vi "Handmatige besturing met druksensoruitlezing Herschreven.vi"() -> ()   [LabVIEW 2024]
uses:
  <vilib>/DAQmx/write.llb/DAQmx Write (Digital 1D Bool NChan 1Samp 1Line).vi
  <vilib>/DAQmx/read.llb/DAQmx Read (Analog 1D DBL NChan 1Samp).vi
  <vilib>/DAQmx/write.llb/DAQmx Write (Analog DBL 1Chan 1Samp).vi
  <vilib>/DAQmx/create/channels.llb/DAQmx Create Channel (AO-Voltage-Basic).vi
  <vilib>/DAQmx/miscellaneous.llb/DAQmx Fill In Error Info.vi
panel:
  out "Waveform Chart":T1(graph)
  out "data":dbl[](array[numeric]) format="%#_6p"
  out "x-y":dbl
  out "Waveform Chart 2":waveform(dbl)[](graph)
  in  "stop":bool
  in  "file path":path
  in  "Analog output pressure regulator":tag="Dev1/ao0"
  in  "Set pressure Hybrid Heart (Bar)":dbl min=0.0 max=1.0 step=0.1
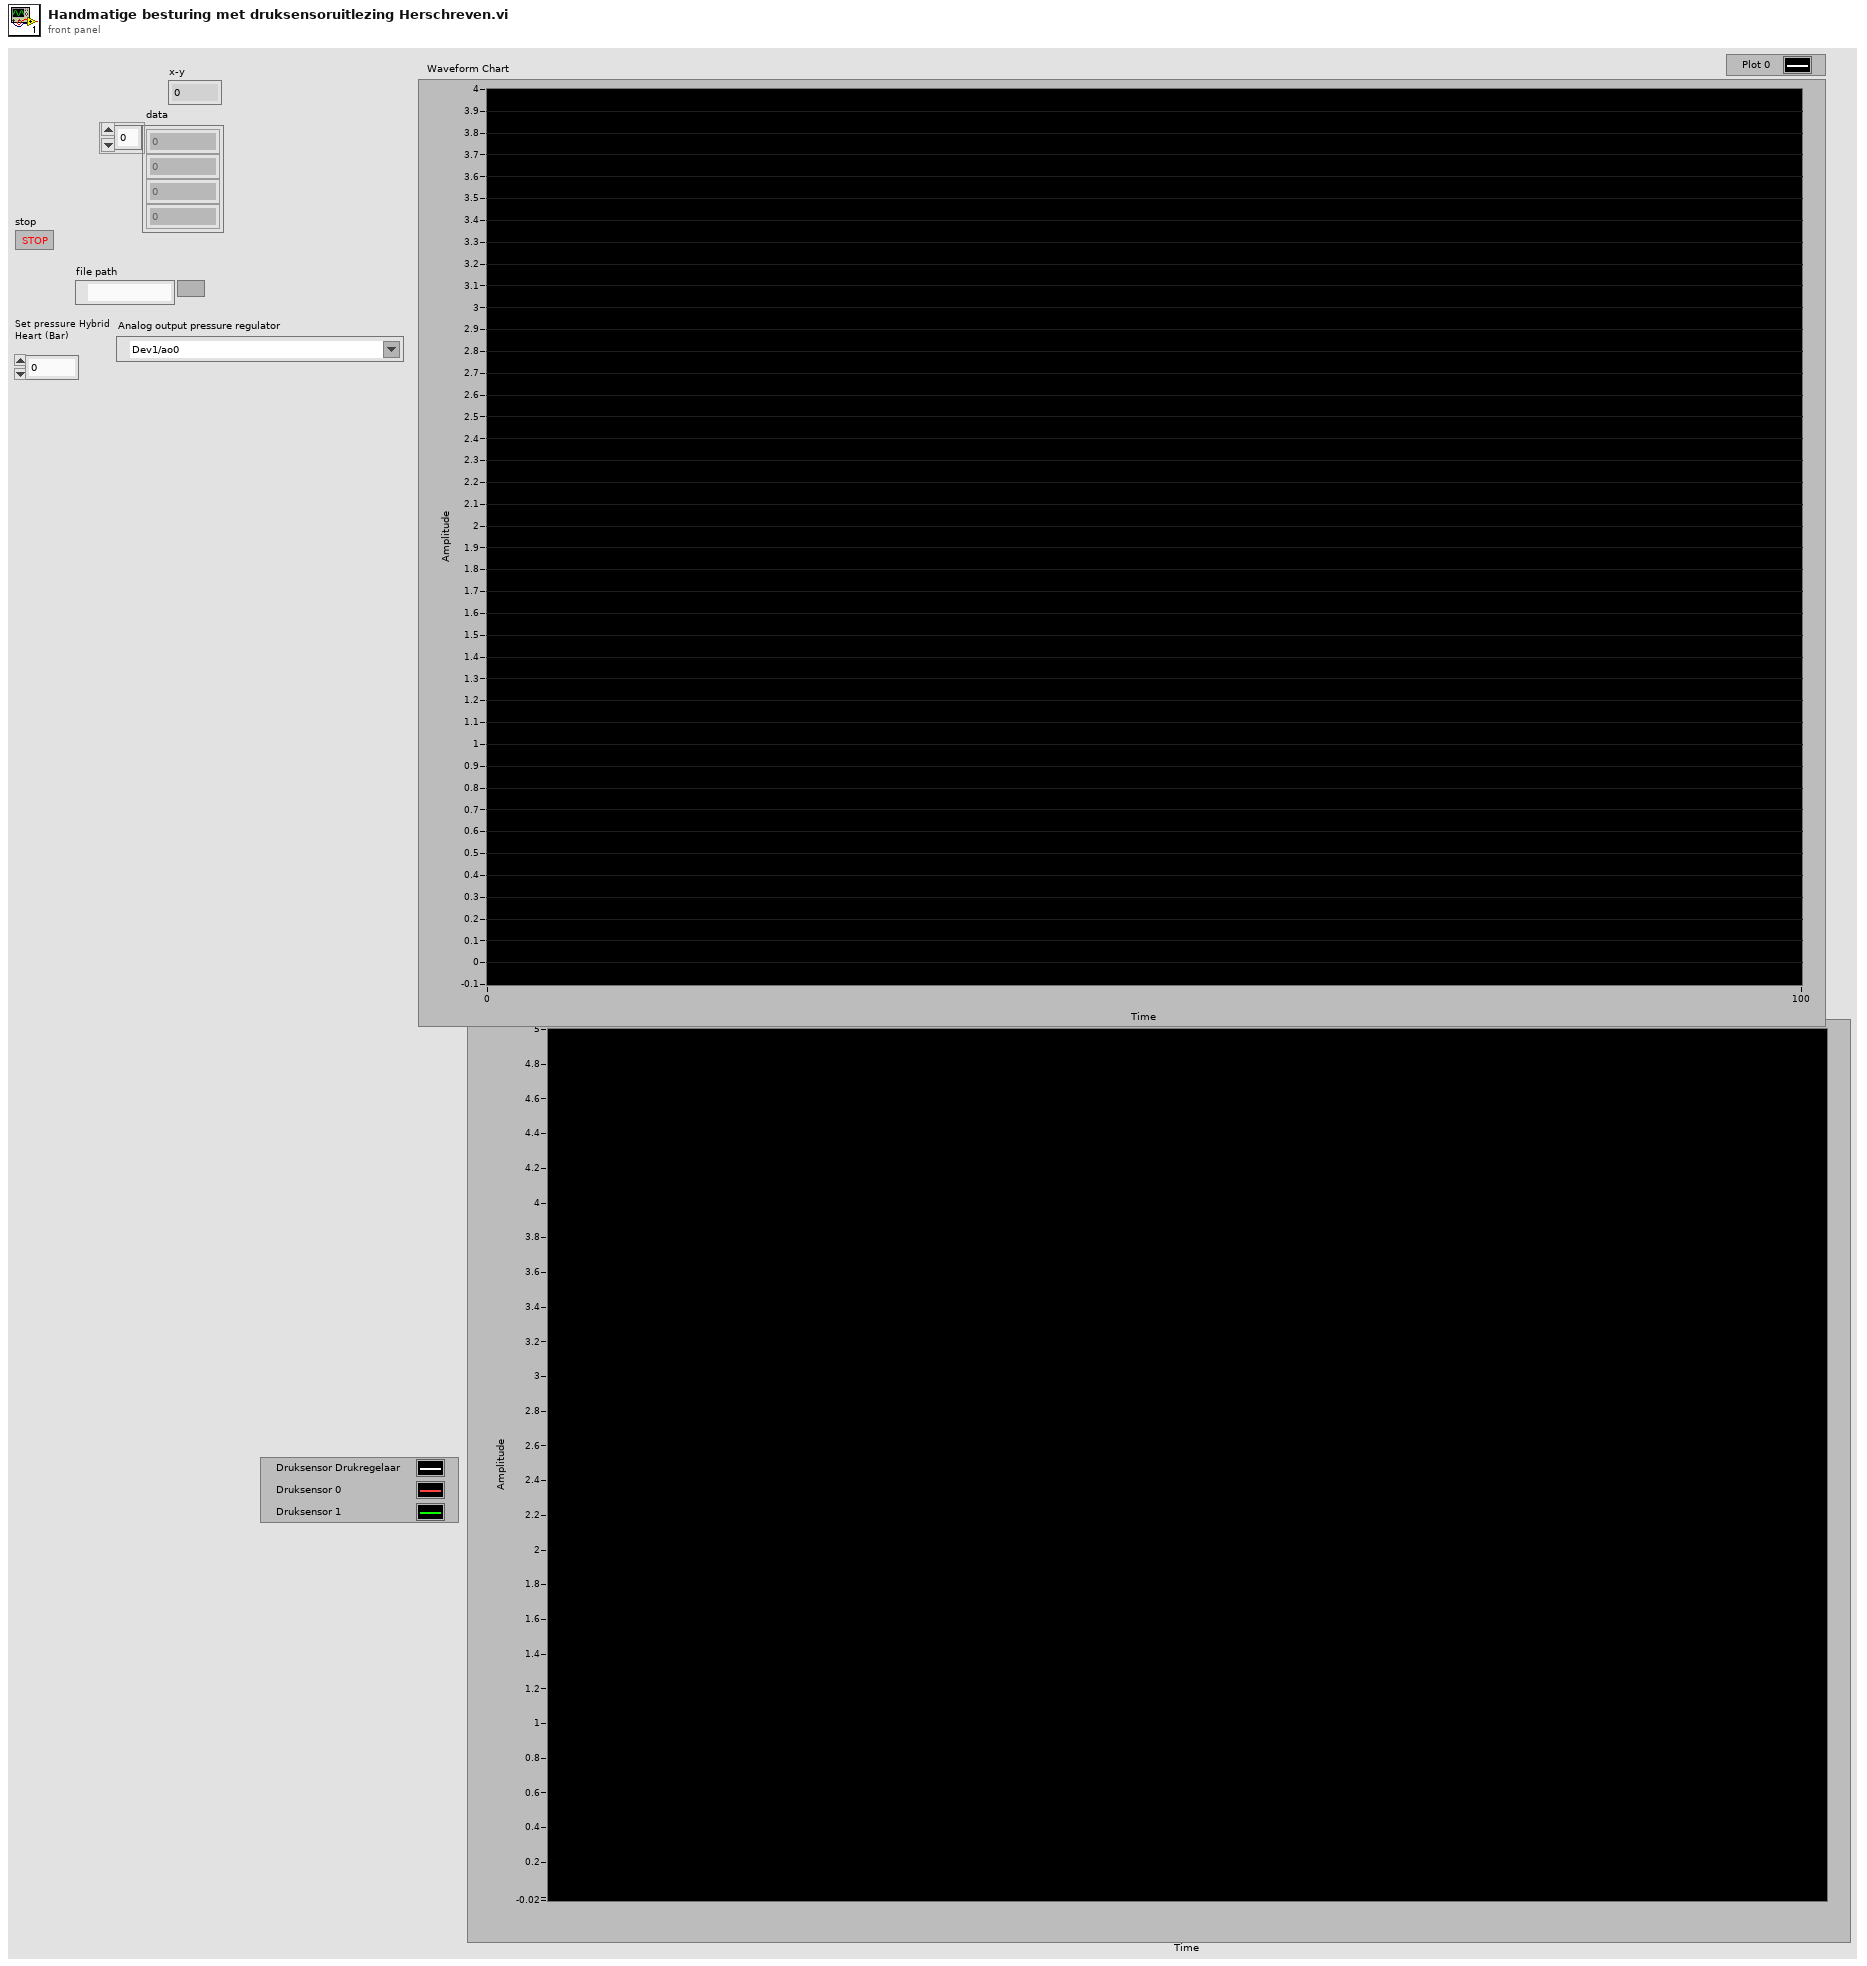
[diagram p1: front panel]
types:
  T1 = cluster{dbl, "Waveform":dbl, "Waveform":dbl, "Waveform":dbl}
  T2 = enum16{"open", "open or create", "create or replace", "create", "open (read-only)"}
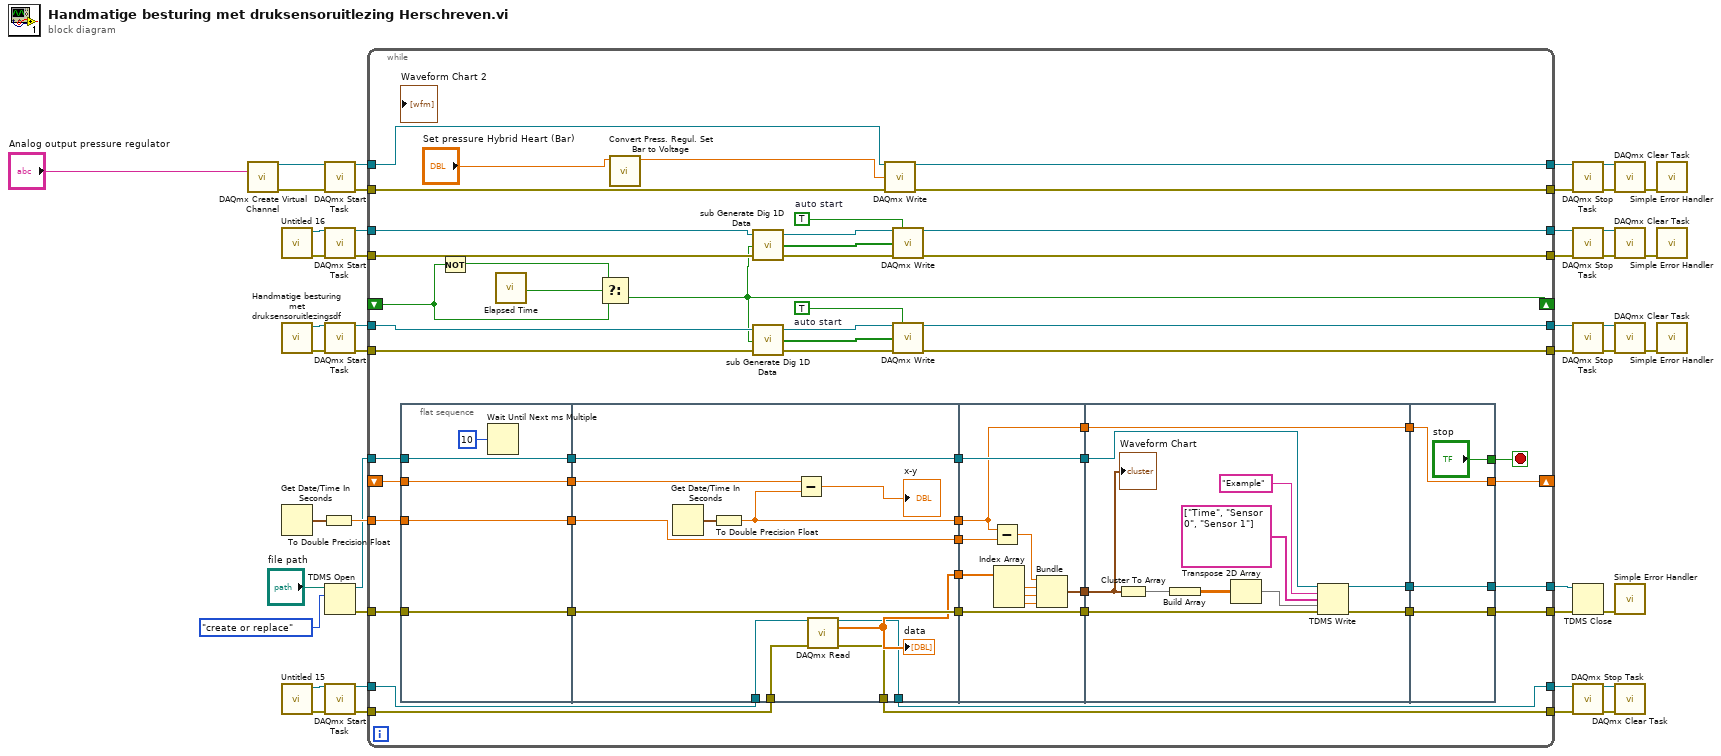
[diagram p0: block diagram]
diagram:
  n1 = call-poly <vilib>:"DAQmx Create Virtual Channel.vi"("physical channels"="Analog output pressure regulator") -> ("task out"=w42:refnum<k21>, "error out"=w41:errorcluster)  [unwired: 13 in]
  n2 = call "Untitled 16.vi"() -> ("error out"=w15:errorcluster, "task out"=w16:refnum<k21>)  [unwired: 10 in]
  n3 = call "Handmatige besturing met druksensoruitlezingsdf.vi"() -> ("error out"=w1:errorcluster, "task out"=w2:refnum<k21>)  [unwired: 10 in]
  n4 = Get Date/Time In Seconds() -> (seconds since 1Jan1904=w34:timestamp)
  n5 = call "Untitled 15.vi"() -> ("error out"=w25:errorcluster, "task out"=w26:refnum<k21>)  [unwired: 10 in]
  n6 = To Double Precision Float(number=w34) -> (double precision float=w33:dbl)
  n7 = call <vilib>:"DAQmx Start Task.vi"("task/channels in"=w42, "error in"=w41) -> ("task out"=w38:refnum<k21>, "error out"=w39:errorcluster)  [unwired: 12 in]
  n8 = call <vilib>:"DAQmx Start Task.vi"("task/channels in"=w16, "error in"=w15) -> ("task out"=w17:refnum<k21>, "error out"=w18:errorcluster)  [unwired: 12 in]
  n9 = call <vilib>:"DAQmx Start Task.vi"("task/channels in"=w2, "error in"=w1) -> ("task out"=w3:refnum<k21>, "error out"=w4:errorcluster)  [unwired: 12 in]
  n10 = TDMS Open(10:T2."create or replace" ("operation (0:open)"), 11:"file path") -> (0:w31:errorcluster, 3:w32:refnum<k34>)  [unwired: 5 in]
  n11 = call <vilib>:"DAQmx Start Task.vi"("task/channels in"=w26, "error in"=w25) -> ("task out"=w24:refnum<k21>, "error out"=w23:errorcluster)  [unwired: 12 in]
  n12 = while {
    tunnel: w38 -> [w97]
    tunnel: w39 -> [w96]
    tunnel: [w95] -> w37
    tunnel: [w94] -> w36
    tunnel: w33 -> [w93]
    tunnel: w32 -> [w89]
    tunnel: w31 -> [w87]
    tunnel: [w84] -> w29
    tunnel: [w83] -> w28
    shift-right: [w75] -> _
    shift-left: _ -> [w71]
    tunnel: [w69] -> w20
    tunnel: [w68] -> w19
    tunnel: w23 -> [w67]
    tunnel: w24 -> [w66]
    tunnel: w4 -> [w57]
    tunnel: w3 -> [w56]
    tunnel: w18 -> [w55]
    tunnel: w17 -> [w54]
    tunnel: [w53] -> w14
    tunnel: [w52] -> w12
    tunnel: [w51] -> w10
    tunnel: [w50] -> w9
    shift-right: [w46] -> _
    shift-left: _ -> [w49]
    stop <- w91 stop-if-true
    w59 = TRUE  # auto start
    w58 = TRUE  # auto start
    n13 = flat-sequence {
      tunnel: [w103] -> w82
      tunnel: w93 -> [w103]
      tunnel: [w102] -> w80
      tunnel: w89 -> [w102]
      tunnel: [w101] -> w78
      tunnel: w87 -> [w101]
      tunnel: [w100] -> w72
      tunnel: w71 -> [w100]
      tunnel: w82 -> [w116]
      tunnel: [w116] -> w81
      tunnel: w80 -> [w115]
      tunnel: [w115] -> w79
      tunnel: w78 -> [w114]
      tunnel: [w114] -> w77
      tunnel: [w111] -> w76
      tunnel: w72 -> [w112]
      tunnel: [w109] -> w70
      tunnel: [w108] -> w69
      tunnel: [w107] -> w68
      tunnel: w67 -> [w106]
      tunnel: w66 -> [w105]
      tunnel: w81 -> [w126]
      tunnel: [w124] -> w92
      tunnel: [w123] -> w90
      tunnel: w79 -> [w123]
      tunnel: [w122] -> w88
      tunnel: w77 -> [w122]
      tunnel: w76 -> [w118]
      tunnel: [w118] -> w73
      tunnel: w70 -> [w117]
      tunnel: w92 -> [w127]
      tunnel: w90 -> [w132]
      tunnel: w88 -> [w131]
      tunnel: [w130] -> w86
      tunnel: [w129] -> w85
      tunnel: [w128] -> w74
      tunnel: w73 -> [w128]
      tunnel: ["stop"] -> w91
      tunnel: [w140] -> w84
      tunnel: w86 -> [w140]
      tunnel: [w139] -> w83
      tunnel: w85 -> [w139]
      tunnel: [w138] -> w75
      tunnel: w74 -> [w138]
      frame #0 {
        n14 = Wait Until Next ms Multiple(millisecond multiple=u32 10) -> ()  [unwired: 1 out]
      }
      frame #1 {
        n15 = Get Date/Time In Seconds() -> (seconds since 1Jan1904=w113:timestamp)
        n16 = To Double Precision Float(number=w113) -> (double precision float=w111:dbl)
        n17 = Subtract(x=w112, y=w111) -> (x-y=→"x-y":dbl)
        n18 = call-poly <vilib>:"DAQmx Read.vi"("task/channels in"=w105, "error in"=w106) -> ("task out"=w108:refnum<k21>, "data"=w109:dbl[], "error out"=w107:errorcluster)  [unwired: 11 in]
        "data" <- w109
      }
      frame #2 {
        n19 = Subtract(x=w118, y=w126) -> (x-y=w125:dbl)
        n20 = Index Array(array=w117) -> (element #1=w121:dbl, element #2=w120:dbl, element #3=w119:dbl)  [unwired: 3 in]
        n21 = Bundle(w125, "Waveform"=w121, "Waveform"=w120, "Waveform"=w119) -> (w124:T1)  [unwired: 1 in]
      }
      frame #3 {
        n22 = Cluster To Array(cluster=w127) -> (array=w137:dbl[])
        n23 = Build Array(w137) -> (w136:dbl[][])
        n24 = Transpose 2D Array(2D array=w136) -> (transposed array=w135:dbl[][])
        n25 = TDMS Write(0:w132, 5:"Example" ("group name in (Untitled)"), 7:string[] ["Time", "Sensor 0", "Sensor 1"] ("channel name(s) in (Untitled)"), 9:w135, 11:w131) -> (4:w129:refnum<k34>, 15:w130:errorcluster)  [unwired: 1 in, 2 out]
        "Waveform Chart" <- w127
      }
      frame #4 {
      }
    }
    n26 = Not(x=w49) -> (.not. x?=w48:bool)
    n27 = call "Elapsed Time"() -> ("Time has Elapsed"=w47:bool)  [unwired: 12 in, 7 out]
    n28 = Select(t=w48, s=w47, f=w49) -> (s? t:f=w46:bool)
    n29 = call "Convert Press. Regul. Set Bar to Voltage.vi"("Set pressure Hybrid Heart (Bar)"="Set pressure Hybrid Heart (Bar)") -> ("Numeric"=w99:dbl)  [unwired: 10 in]
    n30 = call <vilib>:"sub Generate Dig 1D Data.vi"("error in"=w55, "initial value"=w46, "task in"=w54) -> ("error out"=w62:errorcluster, "Data"=w61:bool[], "task out"=w60:refnum<k21>)
    n31 = call <vilib>:"sub Generate Dig 1D Data.vi"("error in"=w57, "initial value"=w46, "task in"=w56) -> ("error out"=w65:errorcluster, "Data"=w64:bool[], "task out"=w63:refnum<k21>)
    n32 = call-poly <vilib>:"DAQmx Write.vi"("task/channels in"=w97, "data"=w99, "error in"=w96) -> ("task out"=w94:refnum<k21>, "error out"=w95:errorcluster)  [unwired: 10 in, 1 out]
    n33 = call-poly <vilib>:"DAQmx Write.vi"("task/channels in"=w60, "auto start"=w59, "data"=w61, "error in"=w62) -> ("task out"=w53:refnum<k21>, "error out"=w52:errorcluster)  [unwired: 9 in, 1 out]
    n34 = call-poly <vilib>:"DAQmx Write.vi"("task/channels in"=w63, "auto start"=w58, "data"=w64, "error in"=w65) -> ("task out"=w51:refnum<k21>, "error out"=w50:errorcluster)  [unwired: 9 in, 1 out]
  }
  n35 = call <vilib>:"DAQmx Stop Task.vi"("task/channels in"=w36, "error in"=w37) -> ("task out"=w44:refnum<k21>, "error out"=w45:errorcluster)  [unwired: 12 in]
  n36 = call <vilib>:"DAQmx Stop Task.vi"("task/channels in"=w14, "error in"=w12) -> ("task out"=w13:refnum<k21>, "error out"=w11:errorcluster)  [unwired: 12 in]
  n37 = call <vilib>:"DAQmx Stop Task.vi"("task/channels in"=w10, "error in"=w9) -> ("task out"=w7:refnum<k21>, "error out"=w8:errorcluster)  [unwired: 12 in]
  n38 = TDMS Close(8:w29, 11:w28) -> (0:w27:errorcluster)  [unwired: 1 out]
  n39 = call <vilib>:"DAQmx Stop Task.vi"("task/channels in"=w20, "error in"=w19) -> ("task out"=w22:refnum<k21>, "error out"=w21:errorcluster)  [unwired: 12 in]
  n40 = call <vilib>:"DAQmx Clear Task.vi"("task in"=w44, "error in"=w45) -> ("error out"=w43:errorcluster)  [unwired: 13 in]
  n41 = call <vilib>:"DAQmx Clear Task.vi"("task in"=w13, "error in"=w11) -> ("error out"=w5:errorcluster)  [unwired: 13 in]
  n42 = call <vilib>:"DAQmx Clear Task.vi"("task in"=w7, "error in"=w8) -> ("error out"=w6:errorcluster)  [unwired: 13 in]
  n43 = call <vilib>:"Simple Error Handler.vi"("error in (no error)"=w27) -> ()  [unwired: 4 in, 5 out]
  n44 = call <vilib>:"DAQmx Clear Task.vi"("task in"=w22, "error in"=w21) -> ()  [unwired: 13 in, 1 out]
  n45 = call <vilib>:"Simple Error Handler.vi"("error in (no error)"=w43) -> ()  [unwired: 4 in, 5 out]
  n46 = call <vilib>:"Simple Error Handler.vi"("error in (no error)"=w5) -> ()  [unwired: 4 in, 5 out]
  n47 = call <vilib>:"Simple Error Handler.vi"("error in (no error)"=w6) -> ()  [unwired: 4 in, 5 out]
